vi "VIH Platform - LabVIEW - VI Property - Help - Use Web Url (2014).vi"(6 "cmd (read)":enum16{"read", "write"}(ring), 8 "error in":errorcluster, 10 "UseWebURL":bool, 11 "VI Refnum":refnum<vi>) -> (0 "error out":errorcluster, 2 "UseWebURL out":bool, 3 "dup VI Refnum":refnum<vi>)   [LabVIEW 2014]
doc: "::: VI Helpeks :::\nCopyright (c) 2000-2026 Konstantin Shifershteyn. All rights reserved."
panel:
  # "VI Helpeks\nCopyright (c) 2012-2026 Konstantin Shifershteyn"
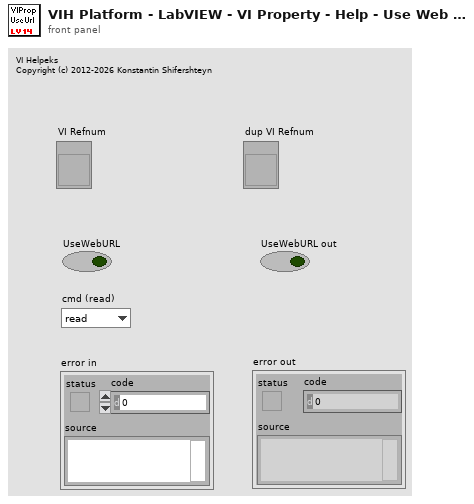
[diagram p1: front panel]
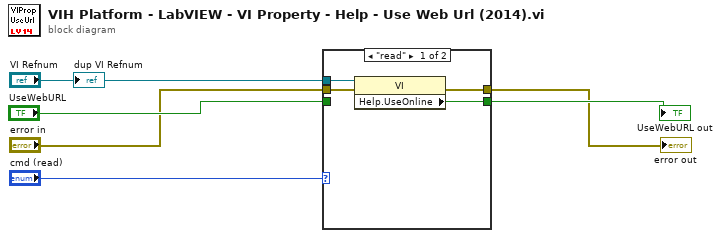
[diagram p0: block diagram]
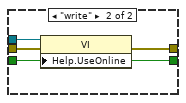
[diagram p2: hidden frame]
diagram:
  n1 = case shown="\"read\"" "cmd (read)" {
    tunnel: "VI Refnum" -> [w10 w14]
    tunnel: "error in" -> [w9 w13]
    tunnel: [w8 w12] -> w1
    tunnel: "UseWebURL" -> [_ w11]
    tunnel: [w7 w11] -> w2
    frame "read" {
      n2 = property class="VI"(reference=w10, error in=w9) -> (error out=w8:errorcluster, "Help.UseOnline"=w7:bool)  [unwired: 1 out]
    }
    frame "write" {
      n3 = property class="VI"(reference=w14, error in=w13, "Help.UseOnline"=w11) -> (error out=w12:errorcluster)  [unwired: 1 out]
    }
  }
  "error out" <- w1
  "UseWebURL out" <- w2
  "dup VI Refnum" <- "VI Refnum"
